vi "Event Handler.vi"(8 "error in (no error)":errorcluster, 10 "Stop Event Handler":refnum<user-event>, 11 "ScrollZoomGraphChart in":refnum<class "ScrollZoomGraphChart.lvclass">) -> (0 "error out":errorcluster)   [LabVIEW 2023, in "TLB` InstStu GPlugin Template.lvlib" / "ScrollZoomGraphChart.lvclass"]
doc: "The <b>Event Handler VI</b> is a dynamic dispatch VI that should be overwritten if events are needed to create the enhanced QControl. \n\nBy inheriting from the main Control.lvclass the overwritten <b>Event Handler VI</b> will be launched asynchronously in the initialization of the QControl.\n<b> </b> <b> </b>\n©2016 Q Software Innovations, LLC (QSI)\nwritten by Quentin Alldredge\nproduced in LabVIEW 2015\n\nsupport@qsoftwareinnovations.com\nwww.qsoftwareinnovations.com\n\nAll rights reserved.\n\nRedistribution and use in source and binary forms, with or without modification, are permitted provided that the following conditions are met:\n\n * Redistributions of source code must retain the above copyright notice, this list of conditions and the following disclaimer.\n * Redistributions in binary form must reproduce the above copyright notice, this list of conditions and the following disclaimer in the documentation and/or other materials provided with the distribution.\n * Neither the name of Q Software Innovations, LLC. nor the names of its contributors may be used to endorse or promote products derived from this software without specific prior written permission.\n\nTHIS SOFTWARE IS PROVIDED BY THE COPYRIGHT HOLDERS AND CONTRIBUTORS \"AS IS\" AND ANY EXPRESS OR IMPLIED WARRANTIES, INCLUDING, BUT NOT LIMITED TO, THE IMPLIED WARRANTIES OF MERCHANTABILITY AND FITNESS FOR A PARTICULAR PURPOSE ARE DISCLAIMED. IN NO EVENT SHALL THE COPYRIGHT OWNER OR CONTRIBUTORS BE LIABLE FOR ANY DIRECT, INDIRECT, INCIDENTAL, SPECIAL, EXEMPLARY, OR CONSEQUENTIAL DAMAGES (INCLUDING, BUT NOT LIMITED TO, PROCUREMENT OF SUBSTITUTE GOODS OR SERVICES; LOSS OF USE, DATA, OR PROFITS; OR BUSINESS INTERRUPTION) HOWEVER CAUSED AND ON ANY THEORY OF LIABILITY, WHETHER IN CONTRACT, STRICT LIABILITY, OR TORT (INCLUDING NEGLIGENCE OR OTHERWISE) ARISING IN ANY WAY OUT OF THE USE OF THIS SOFTWARE, EVEN IF ADVISED OF THE POSSIBILITY OF SUCH DAMAGE."
uses:
  ScrollZoomGraphChart.lvclass
  ScrollZoomGraphChart.lvclass/ScrollZoomGraphChart.ctl
  <vilib>/Analysis/geometry.llb/Point in Polygon Position.ctl
  c12e3cb6-15a2-4a40-9144-b1003a9e759b.vi
  <vilib>/Analysis/geometry.llb/Point in Polygon.vi
  <vilib>/Analysis/geometry.llb/Point in Polygon (Scalar).vi
  <vilib>/Utility/error.llb/Error Cluster From Error Code.vi
  <vilib>/Analysis/NI_AAL_Geometry.lvlib
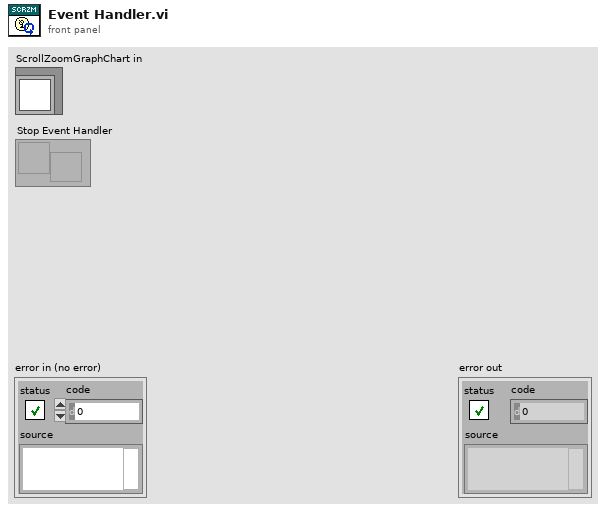
[diagram p1: front panel]
types:
  T1 = typedef "ScrollZoomGraphChart.lvclass/State Data.ctl" = cluster{"X Scales":refnum<vi>[], "Y Scales":refnum<vi>[]}
  T2 = typedef "NI_AAL_Geometry.lvlib/Point in Polygon Position.ctl" = u16
  T3 = typedef "LVPoint32TypeDef.ctl" = cluster{"Horizontal":i32, "Vertical":i32}
  T4 = typedef "LVRectTypeDef.ctl" = cluster{"Left":i16, "Top":i16, "Right":i16, "Bottom":i16}
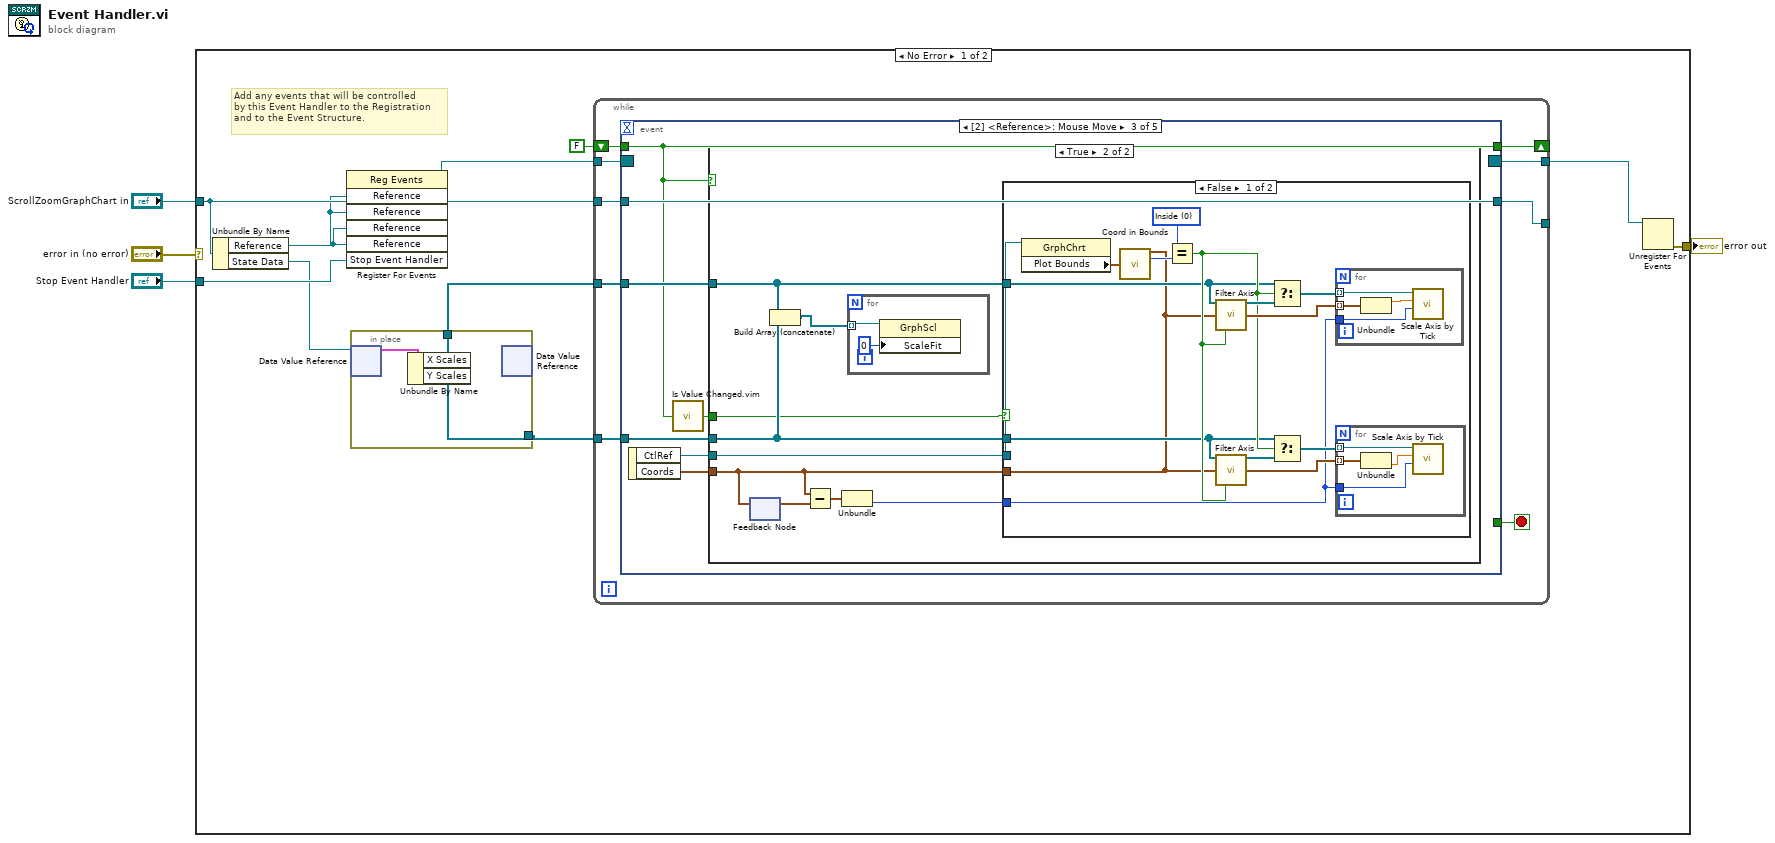
[diagram p0: block diagram]
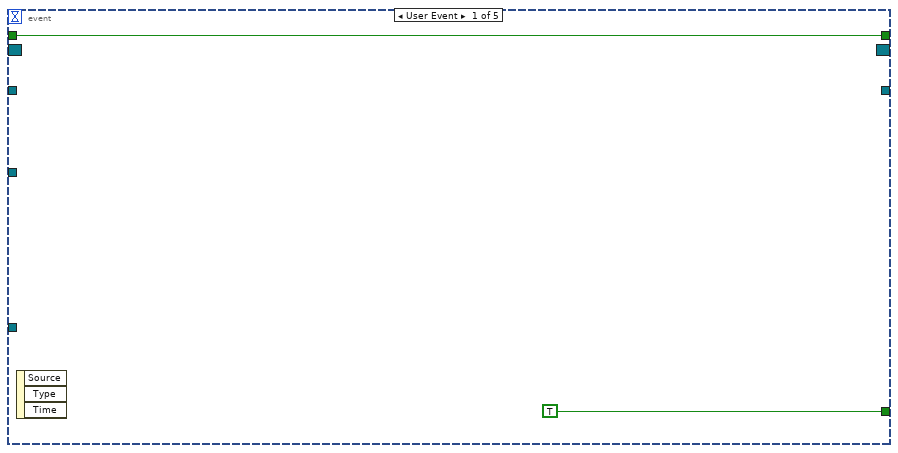
[diagram p2: hidden frame]
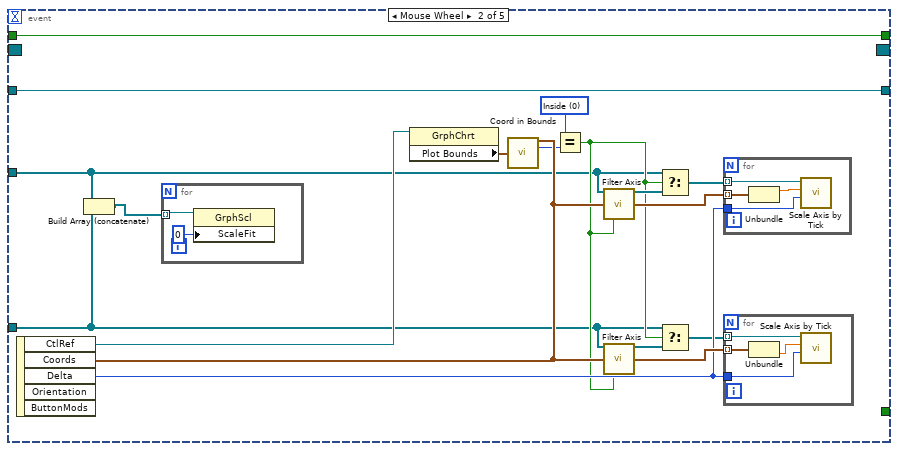
[diagram p3: hidden frame]
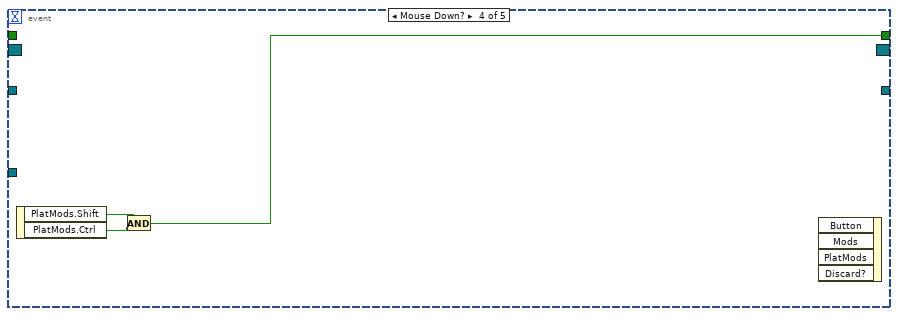
[diagram p6: hidden frame]
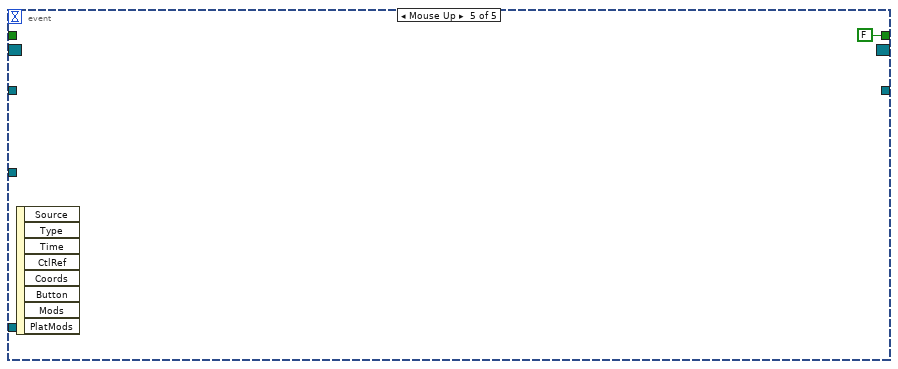
[diagram p7: hidden frame]
diagram:
  n1 = case shown="No Error" "error in (no error)" {
    selector: "error in (no error)" -> [_ w102]
    tunnel: [w14 w102] -> w3
    tunnel: "ScrollZoomGraphChart in" -> [w11 _]
    tunnel: "Stop Event Handler" -> [w13 _]
    frame No Error {
      # "Add any events that will be controlled\nby this Event Handler to the Registration\nand to the Event Structure."
      n2 = Unbundle By Name(w11) -> ("Reference"=w5:refnum<vi>, "State Data"=w10:refnum<data-value>)
      n3 = register-events(w5, w5, w5, w5, w13) -> (reference out=w12:refnum<event-registration>)  [unwired: 2 in, 1 out]
      n4 = in-place {
        in-place-border: [w16] -> w9
        in-place-border: [w15] -> w8
        n5 = in-place-dvr #1(w10) -> (w17:T1)  [unwired: 1 out]
        n6 = Unbundle By Name(w17) -> ("X Scales"=w16:refnum<vi>[], "Y Scales"=w15:refnum<vi>[])
        n7 = in-place-dvr #1() -> ()  [unwired: 1 in, 2 out]
      }
      n8 = while {
        tunnel: w9 -> [w25]
        tunnel: w8 -> [w24]
        tunnel: w12 -> [w23]
        tunnel: [w22] -> _
        tunnel: w11 -> [w21]
        tunnel: [w20] -> w7
        shift-right: [w19] -> _
        shift-left: FALSE -> [w18]
        stop <- w26 stop-if-true
        n9 = event shown="[2] <Reference>: Mouse Move" {
          selector: w23 -> [_ _ _ _ _]
          dyn-events: [_ _ _ _ _] -> w20
          timeout: _ -> [_ _ _ _ _]
          tunnel: [TRUE _ _ _ _] -> w26
          tunnel: w25 -> [_ w32 w60 _ _]
          tunnel: w24 -> [_ w31 w59 _ _]
          tunnel: [_ w33 w61 _ _] -> w22
          tunnel: w21 -> [_ w33 w61 _ _]
          tunnel: [w27 w29 w58 w98 FALSE] -> w19
          tunnel: w18 -> [w27 w29 w58 _ _]
          event User Event {
            n10 = event-data() -> ()  [unwired: 1 in, 3 out]
          }
          event Mouse Wheel {
            w41 = T2 0 items=["Inside", "On Boundary", "Outside"] ("x")
            n11 = event-data() -> ("CtlRef"=w40:refnum<vi>, "Coords"=w43:T3, "Delta"=w37:i32)  [unwired: 1 in, 2 out]
            n12 = Build Array (concatenate)(w32, w31) -> (w30:refnum<vi>[])
            n13 = for {
              tunnel: w30 -> [w48] mode=indexing
              n14 = property class="GrphScl"(reference=w48, "ScaleFit"=u8 0 ("Scale Fit")) -> ()  [unwired: 1 in, 2 out]
            }
            n15 = property class="GrphChrt"(reference=w40) -> ("Plot Bounds"=w44:T4)  [unwired: 1 in, 2 out]
            n16 = call "Coord in Bounds.vi"("Coords"=w43, "Plot Bounds"=w44) -> ("position"=w42:T2)  [unwired: 12 in, 1 out]
            n17 = Equal?(x=w41, y=w42) -> (x = y?=w34:bool)
            n18 = call "Filter Axis.vi"("Graph Scale in"=w32, "Coords"=w43, "Bypass Filter"=w34) -> ("Filter Graph Scale out"=w46:refnum<vi>[], "Axis Value"=w45:cluster{"X":dbl, "Y":dbl}[])  [unwired: 10 in, 1 out]
            n19 = call "Filter Axis.vi"("Graph Scale in"=w31, "Coords"=w43, "Bypass Filter"=w34) -> ("Filter Graph Scale out"=w39:refnum<vi>[], "Axis Value"=w38:cluster{"X":dbl, "Y":dbl}[])  [unwired: 10 in, 1 out]
            n20 = Select(t=w32, s=w34, f=w46) -> (s? t:f=w36:refnum<vi>[])
            n21 = Select(t=w31, s=w34, f=w39) -> (s? t:f=w35:refnum<vi>[])
            n22 = for {
              tunnel: w36 -> [w56] mode=indexing
              tunnel: w45 -> [w55] mode=indexing
              tunnel: w37 -> [w53]
              n23 = Unbundle(w55) -> ("X"=w54:dbl)  [unwired: 1 out]
              n24 = call "Scale Axis by Tick.vi"("Tick Scale"=w53, "Axis Focus Value"=w54, "GraphScale in"=w56) -> ()  [unwired: 9 in]
            }
            n25 = for {
              tunnel: w35 -> [w52] mode=indexing
              tunnel: w38 -> [w51] mode=indexing
              tunnel: w37 -> [w50]
              n26 = Unbundle(w51) -> ("Y"=w49:dbl)  [unwired: 1 out]
              n27 = call "Scale Axis by Tick.vi"("Tick Scale"=w50, "Axis Focus Value"=w49, "GraphScale in"=w52) -> ()  [unwired: 9 in]
            }
          }
          event Mouse Move {
            n28 = event-data() -> ("CtlRef"=w62:refnum<vi>, "Coords"=w63:T3)  [unwired: 1 in]
            n29 = call "Is Value Changed.vim"("value"=w58) -> ("changed or first call?"=w57:bool)
            n30 = case shown="True" w58 {
              tunnel: w63 -> [_ w68]
              tunnel: w62 -> [_ w72]
              tunnel: w60 -> [_ w71]
              tunnel: w59 -> [_ w70]
              tunnel: w57 -> [_ w65]
              frame False {
              }
              frame True {
                n31 = feedback-in #2(w68) -> ()
                n32 = feedback #2() -> (w67:T3)  [unwired: 1 in]
                n33 = Build Array (concatenate)(w71, w70) -> (w69:refnum<vi>[])
                n34 = Subtract(x=w68, y=w67) -> (x-y=w66:T3)
                n35 = Unbundle(w66) -> ("Vertical"=w64:i32)  [unwired: 1 out]
                n36 = for {
                  tunnel: w69 -> [w97] mode=indexing
                  n37 = property class="GrphScl"(reference=w97, "ScaleFit"=u8 0 ("Scale Fit")) -> ()  [unwired: 1 in, 2 out]
                }
                n38 = case shown="False" w65 {
                  tunnel: w72 -> [w82 _]
                  tunnel: w71 -> [w76 _]
                  tunnel: w70 -> [w75 _]
                  tunnel: w68 -> [w74 _]
                  tunnel: w64 -> [w73 _]
                  frame False {
                    w83 = T2 0 items=["Inside", "On Boundary", "Outside"] ("x")
                    n39 = property class="GrphChrt"(reference=w82) -> ("Plot Bounds"=w85:T4)  [unwired: 1 in, 2 out]
                    n40 = call "Coord in Bounds.vi"("Coords"=w74, "Plot Bounds"=w85) -> ("position"=w84:T2)  [unwired: 12 in, 1 out]
                    n41 = Equal?(x=w83, y=w84) -> (x = y?=w77:bool)
                    n42 = call "Filter Axis.vi"("Graph Scale in"=w76, "Coords"=w74, "Bypass Filter"=w77) -> ("Filter Graph Scale out"=w87:refnum<vi>[], "Axis Value"=w86:cluster{"X":dbl, "Y":dbl}[])  [unwired: 10 in, 1 out]
                    n43 = call "Filter Axis.vi"("Graph Scale in"=w75, "Coords"=w74, "Bypass Filter"=w77) -> ("Filter Graph Scale out"=w81:refnum<vi>[], "Axis Value"=w80:cluster{"X":dbl, "Y":dbl}[])  [unwired: 10 in, 1 out]
                    n44 = Select(t=w76, s=w77, f=w87) -> (s? t:f=w79:refnum<vi>[])
                    n45 = Select(t=w75, s=w77, f=w81) -> (s? t:f=w78:refnum<vi>[])
                    n46 = for {
                      tunnel: w79 -> [w95] mode=indexing
                      tunnel: w86 -> [w94] mode=indexing
                      tunnel: w73 -> [w92]
                      n47 = Unbundle(w94) -> ("X"=w93:dbl)  [unwired: 1 out]
                      n48 = call "Scale Axis by Tick.vi"("Tick Scale"=w92, "Axis Focus Value"=w93, "GraphScale in"=w95) -> ()  [unwired: 9 in]
                    }
                    n49 = for {
                      tunnel: w78 -> [w91] mode=indexing
                      tunnel: w80 -> [w90] mode=indexing
                      tunnel: w73 -> [w89]
                      n50 = Unbundle(w90) -> ("Y"=w88:dbl)  [unwired: 1 out]
                      n51 = call "Scale Axis by Tick.vi"("Tick Scale"=w89, "Axis Focus Value"=w88, "GraphScale in"=w91) -> ()  [unwired: 9 in]
                    }
                  }
                  frame True {
                  }
                }
              }
            }
          }
          event Mouse Down? {
            n52 = event-data() -> ("PlatMods.Shift"=w100:bool, "PlatMods.Ctrl"=w99:bool)  [unwired: 1 in]
            n53 = And(x=w100, y=w99) -> (x .and. y?=w98:bool)
            n54 = event-data() -> ()  [unwired: 5 in, 1 out]
          }
          event Mouse Up {
            n55 = event-data() -> ()  [unwired: 1 in, 8 out]
          }
        }
      }
      n56 = Unregister For Events(event registration refnum=w7) -> (error out=w14:errorcluster)  [unwired: 1 in]
    }
    frame Error {
    }
  }
  "error out" <- w3
